vi "Base species number count.vi"(8 "Signal Sequence":string[](array[string]), 11 "Base Ex Info":T1) -> (0 "All":bool[](array[boolean]), 1 "Base Species C":i32[][](array[numeric]), 2 "b comb":u32[](array[numeric]), 3 "Base Species#":i16[](array[numeric]))   [LabVIEW 2018]
panel:
  out "Base Composition":string[](array[string])
  out "配列 3":i16[][](array[numeric])
  out "配列 4":bool[][](array[boolean])
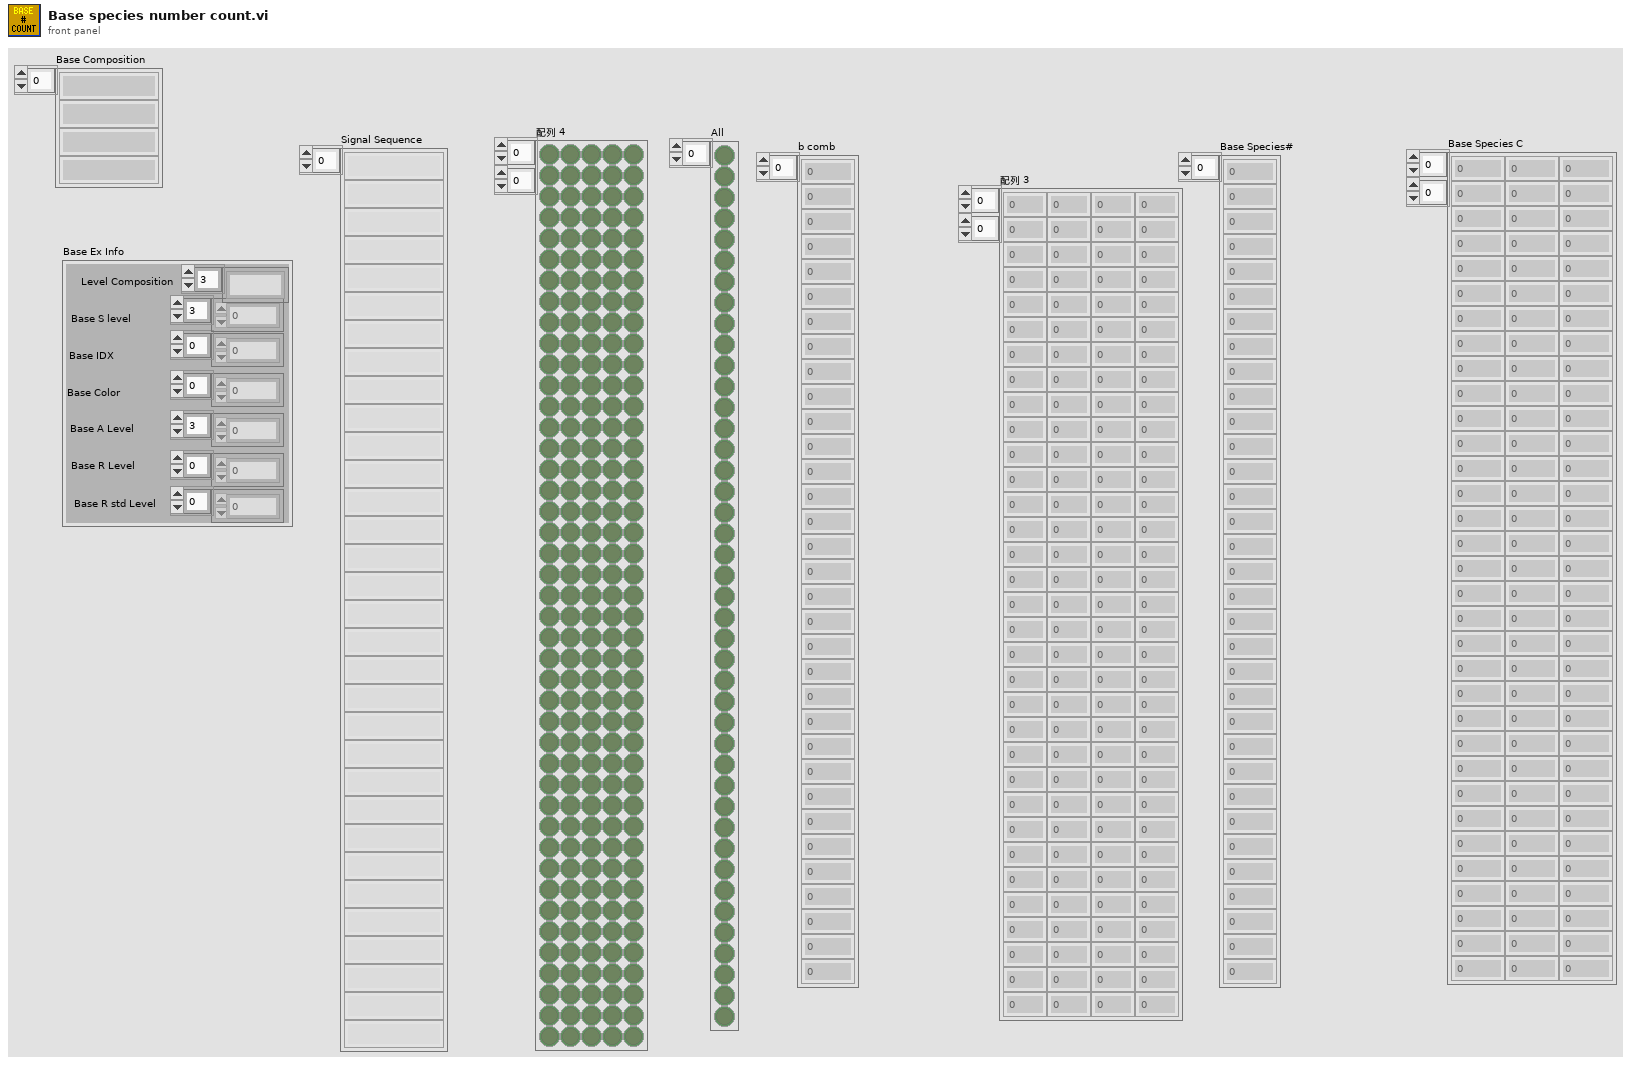
[diagram p1: front panel]
types:
  T1 = cluster{"Level Composition":string[], "Base S level":dbl[], "Base IDX":i32[], "Base Color":u32[], "Base A Level":dbl[], "Base R Level":dbl[], "Base R std Level":dbl[]}
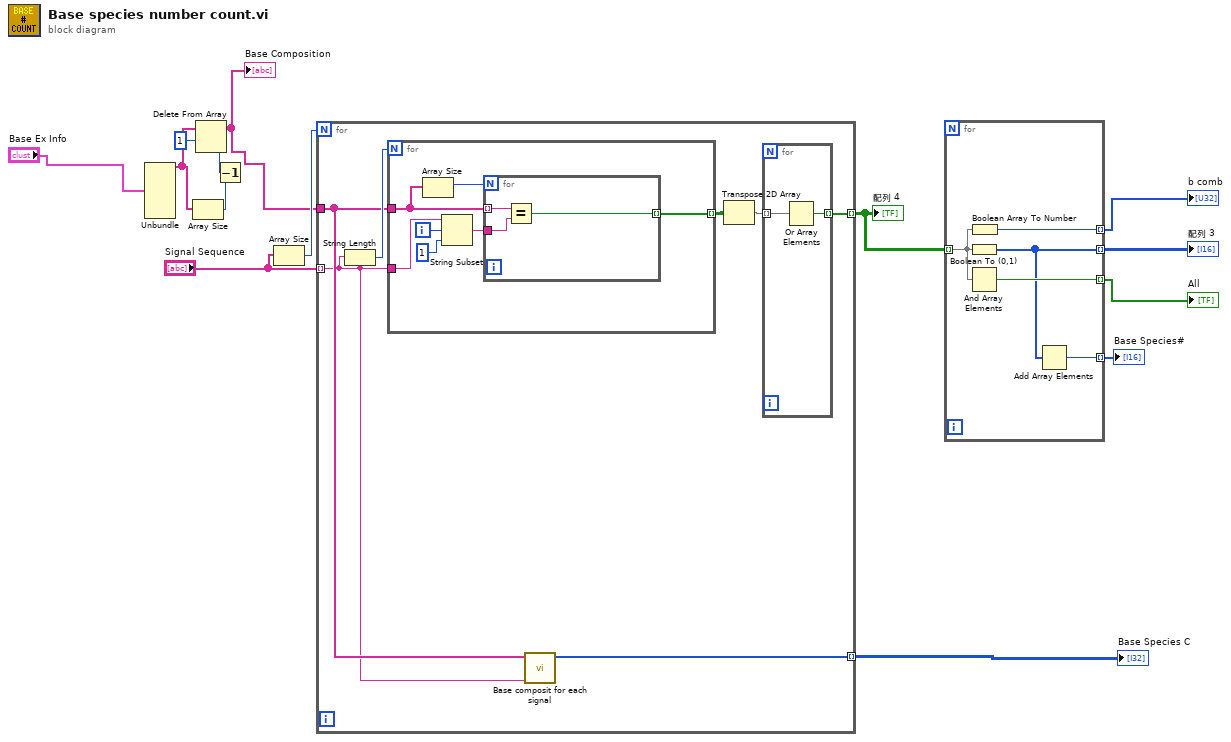
[diagram p0: block diagram]
diagram:
  n1 = Unbundle("Base Ex Info") -> ("Level Composition"=w6:string[])  [unwired: 6 out]
  n2 = Array Size(array=w6) -> (size(s)=w5:i32)
  n3 = Decrement(x=w5) -> (x-1=w4:i32)
  n4 = Delete From Array(array=w6, length=1 ("長さ"), index=w4) -> (array with subset deleted=w3:string[])  [unwired: 1 out]
  "Base Composition" <- w3
  n5 = Array Size(array="Signal Sequence") -> (size(s)=w13:i32)
  n6 = for {
    N: w13 -> [_]
    tunnel: "Signal Sequence" -> [w16] mode=indexing
    tunnel: w3 -> [w17]
    tunnel: [w18] -> w9 mode=indexing
    tunnel: [w15] -> w2 mode=indexing
    n7 = String Length(string=w16) -> (length=w21:i32)
    n8 = for {
      N: w21 -> [_]
      tunnel: w17 -> [w24]
      tunnel: w16 -> [w26]
      tunnel: [w27] -> w19 mode=indexing
      i -> [w28]
      n9 = Array Size(array=w24) -> (size(s)=w30:i32)
      n10 = String Subset(string=w26, offset (0)=w28, length (rest)=1 ("長さ（残り）")) -> (substring=w25:string)
      n11 = for {
        N: w30 -> [_]
        tunnel: w24 -> [w33] mode=indexing
        tunnel: w25 -> [w32]
        tunnel: [w31] -> w27 mode=indexing
        n12 = Equal?(x=w33, y=w32) -> (x = y?=w31:bool)
      }
    }
    n13 = call "Base composit for each signal.vi"("文字列"=w16, "Base Composition"=w17) -> ("Base C"=w15:i32[])  [unwired: 9 in]
    n14 = Transpose 2D Array(2D array=w19) -> (transposed array=w20:bool[][])
    n15 = for {
      tunnel: w20 -> [w23] mode=indexing
      tunnel: [w22] -> w18 mode=indexing
      n16 = Or Array Elements(Boolean array=w23) -> (logical OR=w22:bool)
    }
  }
  "配列 4" <- w9
  "Base Species C" <- w2
  n17 = for {
    tunnel: w9 -> [w36] mode=indexing
    tunnel: [w38] -> w12 mode=indexing
    tunnel: [w37] -> w11 mode=indexing
    tunnel: [w35] -> w10 mode=indexing
    tunnel: [w34] -> w8 mode=indexing
    n18 = Boolean To (0,1)(Boolean=w36) -> (0, 1=w35:i16[])
    n19 = And Array Elements(Boolean array=w36) -> (logical AND=w38:bool)
    n20 = Boolean Array To Number(Boolean array=w36) -> (number=w37:u32)
    n21 = Add Array Elements(numeric array=w35) -> (sum=w34:i16)
  }
  "All" <- w12
  "b comb" <- w11
  "配列 3" <- w10
  "Base Species#" <- w8
